vi "Initialize.vi"(4 "error in (no error)":errorcluster, 7 "Engine Reference":refnum<k7>) -> (0 "error out":errorcluster, 3 "EasyUserManager out":refnum<class "EasyUserManager.lvclass">)   [LabVIEW 2024, in "EasyUserManager.lvclass"]
doc: "Create a new <B>EasyUserManager</B> object instance and set the provided Teststand Engine to the class attribute."
uses:
  EasyUserManager.lvclass
  EasyUserManager.lvclass/EasyUserManager.ctl
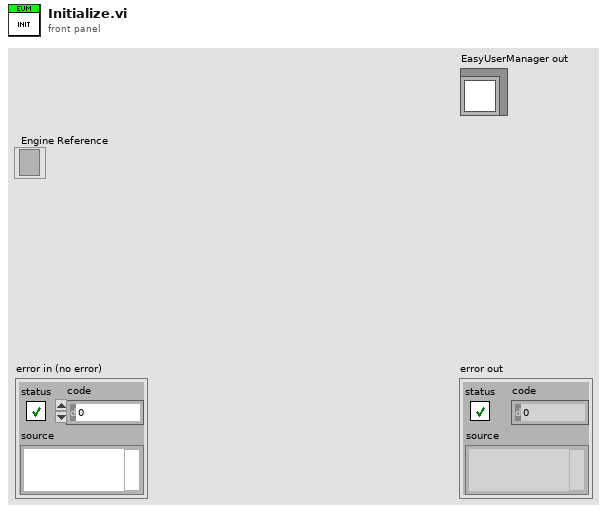
[diagram p1: front panel]
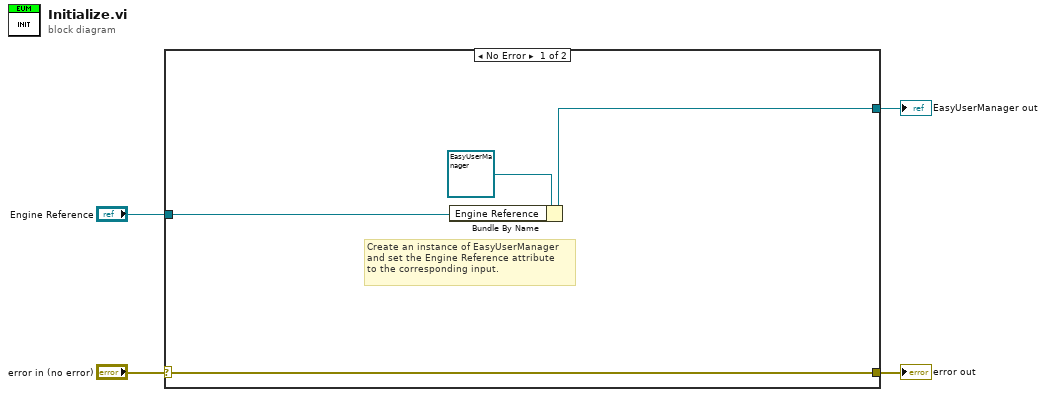
[diagram p0: block diagram]
diagram:
  n1 = case shown="No Error" "error in (no error)" {
    selector: "error in (no error)" -> [w5 w9]
    tunnel: [w5 w9] -> w3
    tunnel: [w8 _] -> w2
    tunnel: "Engine Reference" -> [w6 _]
    frame No Error {
      # "Create an instance of EasyUserManager\nand set the Engine Reference attribute\nto the corresponding input."
      n2 = Bundle By Name(cluster=refnum<class "EasyUserManager.lvclass"> refnum ("EasyUserManager.lvclass"), "Engine Reference"=w6) -> (w8:refnum<class "EasyUserManager.lvclass">)
    }
    frame Error {
      # "Pass error and do nothing."
    }
  }
  "error out" <- w3
  "EasyUserManager out" <- w2
